vi "Get Client Machine Details.vi"(8 "error in":errorcluster) -> (0 "error out":errorcluster, 1 "ip address":string, 2 "username":string, 3 "hostname":string)   [LabVIEW 2021, in "NI Session Management V1 Client.lvlib" / "Session Reservation.lvclass"]
uses:
  Session Reservation.lvclass
  kernel32.dll
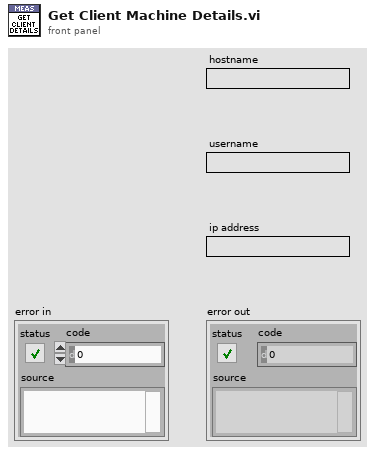
[diagram p1: front panel]
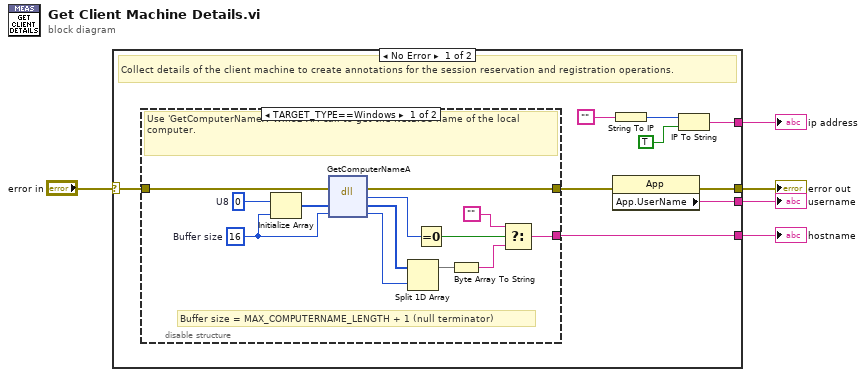
[diagram p0: block diagram]
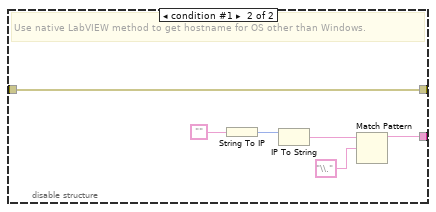
[diagram p2: hidden frame]
diagram:
  n1 = case shown="No Error" "error in" {
    selector: "error in" -> [w8 w34]
    tunnel: [w12 w34] -> w4
    tunnel: [w13 _] -> w5
    tunnel: [w6 _] -> w3
    tunnel: [w11 _] -> w1
    frame No Error {
      # "Collect details of the client machine to create annotations for the session reservation and registration operations."
      n2 = disable-structure shown="TARGET_TYPE==Windows" {
        disable-tunnel: w8 -> [w27 w33]
        disable-tunnel: [w23 w33] -> w10
        disable-tunnel: [w22 w29] -> w6
        frame condition #0 (active) {
          w16 = u8 0  # U8
          w15 = u32 16  # Buffer size
          # "Buffer size = MAX_COMPUTERNAME_LENGTH + 1 (null terminator)"
          # "Use 'GetComputerNameA' Win32 API call to get the NetBIOS name of the local computer."
          n3 = Initialize Array(w16, w15) -> (w21:u8[])
          n4 = dll-call lib="kernel32.dll" fn="GetComputerNameA"(error in=w27, "lpBuffer"=w21, "nSize"=w15) -> (error out=w23:errorcluster, "return type"=w24:i32, "lpBuffer"=w26:u8[], "nSize"=w25:u32)  [unwired: 2 in, 1 out]
          n5 = Split 1D Array(array=w26, index=w25) -> (first subarray=w19:u8[])  [unwired: 1 out]
          n6 = Equal To 0?(x=w24) -> (x = 0?=w20:bool)
          n7 = Byte Array To String(unsigned byte array=w19) -> (string=w18:string)
          n8 = Select(t="", s=w20, f=w18) -> (s? t:f=w22:string)
        }
        frame condition #1 {
          # "Use native LabVIEW method to get hostname for OS other than Windows."
          n9 = String To IP(1:"") -> (0:w32:u32)
          n10 = IP To String(2:w32) -> (0:w30:string)  [unwired: 1 in]
          n11 = Match Pattern(string=w30, regular expression="\\.") -> (before substring=w29:string)  [unwired: 1 in, 3 out]
        }
      }
      n12 = property class="App"(error in=w10) -> (error out=w12:errorcluster, "App.UserName"=w11:string)  [unwired: 1 in, 1 out]
      n13 = String To IP(1:"") -> (0:w14:u32)
      n14 = IP To String(1:TRUE ("dot notation? (F)"), 2:w14) -> (0:w13:string)
    }
    frame Error {
    }
  }
  "ip address" <- w5
  "username" <- w1
  "error out" <- w4
  "hostname" <- w3
